vi "Prepare.vi"(8 "error in (no error)":errorcluster, 11 "CIFPlugin in":refnum<class "CAN_Reader_NIXNET_Plugin.lvclass">) -> (0 "error out":errorcluster, 3 "CIFPlugin out":refnum<class "CAN_Reader_NIXNET_Plugin.lvclass">)   [LabVIEW 2021, in "CAN_Reader_NIXNET_Plugin.lvclass"]
uses:
  CAN_Reader_NIXNET_Plugin.lvclass
  CAN_Reader_NIXNET_Plugin.lvclass/CAN_Reader_NIXNET_Plugin.ctl
  <vilib>/CIF Foundation/CIF CAN RW Core/CAN_RW_CORE.lvclass/CAN_RW_CORE.ctl
  <vilib>/CIF Foundation/CIF XNET CAN RW/XNET CAN RW.lvclass
  C:/Program Files/National Instruments/LabVIEW 2021/vi.lib/CIF Foundation/CIF CAN RW Core/CAN_RW_CORE.lvclass
  <vilib>/CIF Foundation/CIF CAN RW Core/CAN_RW_CORE.lvclass
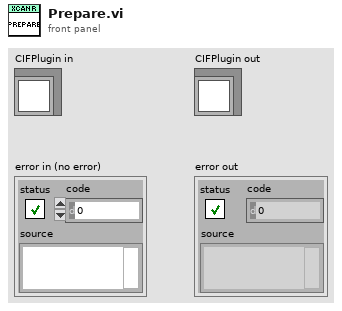
[diagram p1: front panel]
types:
  T1 = typedef "CAN_RW_CORE.lvclass/CAN Port Configuration.ctl" = cluster{"Mode":T2, "Baud Rate":u64, "Temination On":bool, "Subordinate":bool, "Echo TX":bool, "FD Config":T3}
  T2 = typedef "CAN_RW_CORE.lvclass/CAN Mode.ctl" = enum16{"CAN 2.0", "CAN FD"}
  T3 = typedef "CAN_RW_CORE.lvclass/FD Config.ctl" = cluster{"FD Baud Rate":u64, "ISO Mode":bool, "BRS Enabled":bool}
  T4 = typedef "CAN_RW_CORE.lvclass/CAN Filter.ctl" = cluster{"Allow List (ID)":u32[], "Deny List (ID)":u32[]}
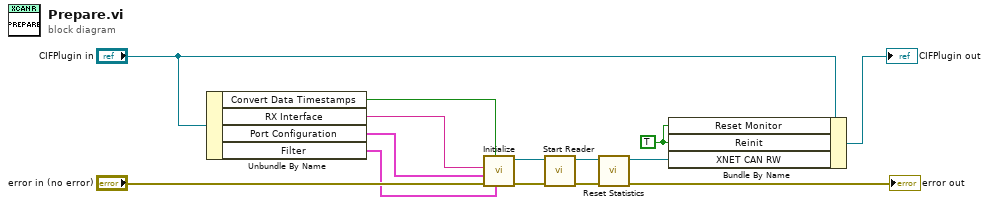
[diagram p0: block diagram]
diagram:
  w5 = TRUE ("External Clock Controls.Reinit")
  n1 = Unbundle By Name("CIFPlugin in") -> ("Convert Data Timestamps"=w9:bool, "RX Interface"=w8:string, "Port Configuration"=w7:T1, "Filter"=w6:T4)
  n2 = call <vilib>:"Initialize.vi"("Filter"=w6, "Use OS Timestamp"=w9, "error in (no error)"="error in (no error)", "Port Configuration"=w7, "Interface"=w8) -> ("error out"=w13:errorcluster, "XNET_CAN_RW out"=w12:refnum<class "XNET CAN RW.lvclass">)  [unwired: 5 in]
  n3 = call-dynamic "Start Reader.vi"("error in (no error)"=w13, "XNET_CAN_RW in"=w12) -> ("error out"=w3:errorcluster, "XNET_CAN_RW out"=w4:refnum<class "XNET CAN RW.lvclass">)  [unwired: 8 in]
  n4 = call <vilib>:"Reset Statistics.vi"("error in (no error)"=w3, "CAN_RW_CORE in"=w4) -> ("error out"=→"error out":errorcluster, "CAN_RW_CORE out"=w2:refnum<class "XNET CAN RW.lvclass">)  [unwired: 8 in]
  n5 = Bundle By Name(cluster="CIFPlugin in", "Reset Monitor"=w5, "Reinit"=w5, "XNET CAN RW"=w2) -> (→"CIFPlugin out":refnum<class "CAN_Reader_NIXNET_Plugin.lvclass">)
